vi "WPI_RobotDriveMecanumMotors.vi"(6 "Rear Right":dbl, 7 "Rear Left":dbl, 8 "error in":errorcluster, 9 "Front Right":dbl, 10 "Front Left":dbl, 11 "RobotDriveDevRef in":T1) -> (0 "error out":errorcluster, 2 "Motor Values":dbl[](array[numeric]), 3 "RobotDriveDevRef out":T1)   [LabVIEW 2023]
doc: "Update each motor with the appropriate power for that wheel."
uses:
  <vilib>/REVLibDriver/REVLibDriver.lvlib
  <vilib>/REV Custom Controls/Spark Output Control Type.ctl
  <vilib>/Rock Robotics/WPI/RobotDrive/WPI_RobotDriveDevRef.ctl
  <vilib>/REV Custom Controls/REVSparkRefnum.ctl
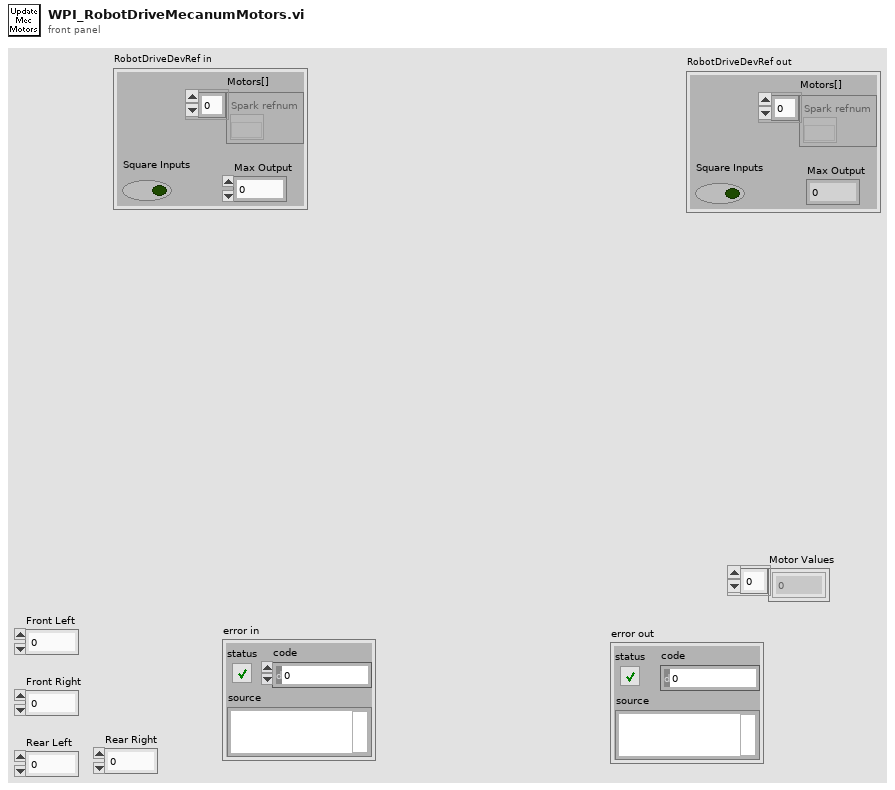
[diagram p1: front panel]
types:
  T1 = typedef "WPI_RobotDriveDevRef.ctl" = cluster{"Motors[]":T2[], "Square Inputs":bool, "Max Output":dbl}
  T2 = typedef "REVLibDriver.lvlib/REVSparkRefnum.ctl" = refnum<k20>
  T3 = typedef "REVLibDriver.lvlib/Spark Output Control Type.ctl" = enum16{"Percent VBus", "Velocity", "Voltage", "Position", "Current", "MAXMotion Position", "MAXMotion Velocity"}
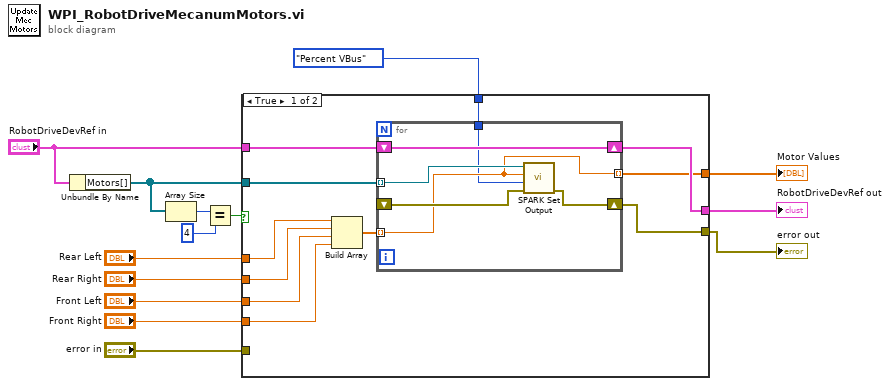
[diagram p0: block diagram]
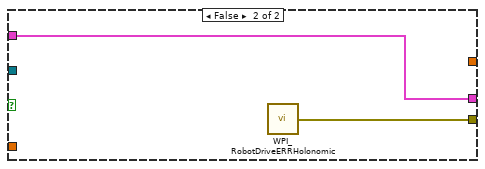
[diagram p2: hidden frame]
diagram:
  n1 = Unbundle By Name("RobotDriveDevRef in") -> ("Motors[]"=w3:T2[])
  n2 = Array Size(array=w3) -> (size(s)=w10:i32)
  n3 = Equal?(x=w10, y=4) -> (x = y?=w12:bool)
  n4 = case shown="True" w12 {
    tunnel: "Front Left" -> [w22 _]
    tunnel: "Front Right" -> [w21 _]
    tunnel: [w18 w33] -> w2
    tunnel: "Rear Left" -> [w24 _]
    tunnel: "Rear Right" -> [w23 _]
    tunnel: [w17 _] -> w13
    tunnel: "error in" -> [_ _]
    tunnel: [w19 w32] -> w14
    tunnel: "RobotDriveDevRef in" -> [w20 w32]
    tunnel: w3 -> [w16 _]
    tunnel: Spark_Output_Control_Type."Percent VBus" ("Control Mode") -> [w15 _]
    frame True {
      n5 = Build Array(w24, w23, w22, w21) -> (w25:dbl[])
      n6 = for {
        tunnel: [w27] -> w17 mode=indexing
        shift-right: [w28] -> w18
        shift-left: _ -> [w29]
        shift-right: [w31] -> w19
        shift-left: w20 -> [w31]
        tunnel: w16 -> [w30] mode=indexing
        tunnel: w25 -> [w27] mode=indexing
        tunnel: w15 -> [w26]
        n7 = call <vilib>:"SPARK Set Output.vi"("error in (no error)"=w29, "Control Mode"=w26, "Setpoint"=w27, "Spark refnum"=w30) -> ("error out"=w28:errorcluster)  [unwired: 6 in, 1 out]
      }
    }
    frame False {
      n8 = call <vilib>:"WPI_RobotDriveERRHolonomic.vi"() -> ("error out"=w33:errorcluster)
    }
  }
  "RobotDriveDevRef out" <- w14
  "error out" <- w2
  "Motor Values" <- w13
